vi "Run Tests.vi"(8 "error in (no error)":errorcluster, 10 "Test Cases":refnum<class "Test Case.lvclass">[](array[class]), 11 "LVUnit Test Executor in":refnum<class "LVUnit Test Executor.lvclass">) -> (0 "error out":errorcluster, 2 "Test Results":refnum<class "Test Result.lvclass">[](array[class]), 3 "LVUnit Test Executor out":refnum<class "LVUnit Test Executor.lvclass">)   [LabVIEW 2017, in "LVUnit Test Executor.lvclass"]
doc: "Runs the specified tests."
uses:
  LVUnit Test Executor.lvclass
  C:/Users/pasca/Projects/Home/lvunit/Test Executor/Test Executor.lvclass
  Test Case/Test Case.lvclass
  Test Result/Test Result.lvclass
  Test Outcome.ctl
  <vilib>/Utility/error.llb/DialogType.ctl
  Test Executor/Test Executor.lvclass/Test Executor.ctl
  Test Case/Test Case.lvclass/Test Case.ctl
  LVUnit Test Case/LVUnit Test Case.lvclass/LVUnit Test Case.ctl
  Test Result/Test Result.lvclass/Test Result.ctl
  Test Case/Get Path.vi
  LVUnit Test Case/Get JSON Data.vi
  Test Result/Set Outcome.vi
  Test Result/Set Failure Message.vi
  Test Result/Set Start Time.vi
  Test Result/Set End Time.vi
  Test Executor/Read Application.vi
  Test Executor/Read Result Queue.vi
  LVUnit Test Case/LVUnit Test Case.lvclass
  C:/Users/pasca/Projects/Home/lvunit/Test Case/Test Case.lvclass
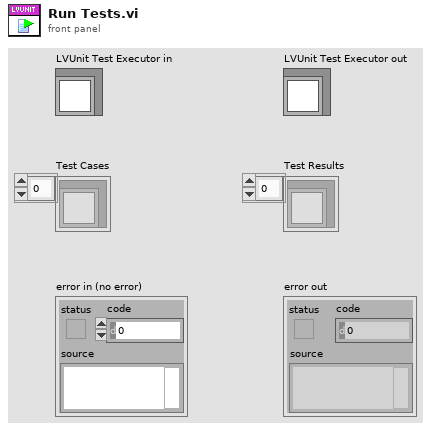
[diagram p1: front panel]
types:
  T1 = typedef "Test Outcome.ctl" = enum16{"None", "Passed", "Failed"}
  T2 = typedef "DialogType.ctl" = u16
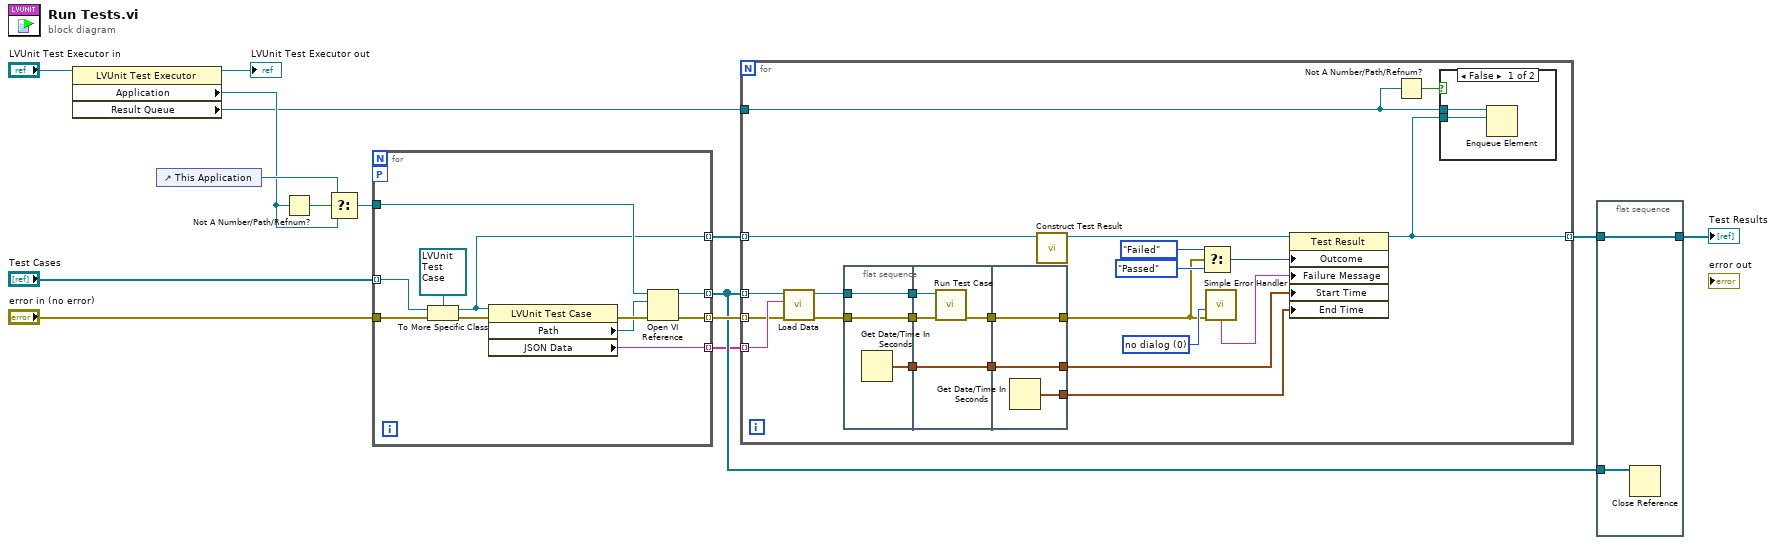
[diagram p0: block diagram]
diagram:
  n1 = property class="LVUnit Test Executor"(reference="LVUnit Test Executor in") -> (reference out=→"LVUnit Test Executor out":refnum<class "LVUnit Test Executor.lvclass">, "Application"=w11:refnum<vi>, "Result Queue"=w1:refnum<queue>)  [unwired: 1 in, 1 out]
  n2 = control-ref of="This Application"() -> (w12:refnum<vi>)
  n3 = Not A Number/Path/Refnum?(number/path/refnum=w11) -> (NaN/Path/Refnum?=w13:bool)
  n4 = Select(t=w12, s=w13, f=w11) -> (s? t:f=w8:refnum<vi>)
  n5 = for {
    tunnel: "Test Cases" -> [w22] mode=indexing
    tunnel: "error in (no error)" -> [w21]
    tunnel: w8 -> [w20]
    tunnel: [w19] -> w7 mode=indexing
    tunnel: [w18] -> w6 mode=indexing
    tunnel: [w17] -> w4 mode=indexing
    workers-P: _ -> [_]
    tunnel: [w16] -> w3 mode=indexing
    n6 = To More Specific Class(target class=refnum<class "LVUnit Test Case.lvclass"> refnum ("LVUnit Test Case.lvclass"), reference=w22, error in=w21) -> (specific class reference=w19:refnum<class "LVUnit Test Case.lvclass">, error out=w25:errorcluster)
    n7 = property class="LVUnit Test Case"(reference=w19, error in=w25) -> (error out=w24:errorcluster, "Path"=w23:path, "JSON Data"=w16:string)  [unwired: 1 out]
    n8 = Open VI Reference(application reference (local)=w20, vi path=w23, error in (no error)=w24) -> (vi reference=w17:refnum<vi>, error out=w18:errorcluster)  [unwired: 3 in]
  }
  n9 = for {
    tunnel: w7 -> [w30] mode=indexing
    tunnel: w6 -> [w40] mode=indexing
    tunnel: w4 -> [w42] mode=indexing
    tunnel: w3 -> [w41] mode=indexing
    tunnel: [w27] -> w2 mode=indexing
    tunnel: w1 -> [w28]
    w34 = T2 0 items=["no dialog", "OK message", "continue or stop message", "OK message + warnings", "continue/stop + warnings"] ("type of dialog (OK msg:1)")
    n10 = call "Load Data.vi"("error in (no error)"=w40, "JSON Data"=w41, "VI Reference"=w42) -> ("error out"=w49:errorcluster, "VI Refnum out"=w43:refnum<vi>)  [unwired: 7 in]
    n11 = flat-sequence {
      tunnel: w43 -> [w53]
      tunnel: w49 -> [w54]
      tunnel: [w54] -> w48
      tunnel: [w53] -> w47
      tunnel: [w52] -> w44
      tunnel: w48 -> [w57]
      tunnel: w47 -> [w56]
      tunnel: [w58] -> w46
      tunnel: [w55] -> w45
      tunnel: w44 -> [w55]
      tunnel: [w61] -> w33
      tunnel: w46 -> [w61]
      tunnel: [w60] -> w32
      tunnel: w45 -> [w60]
      tunnel: [w59] -> w31
      frame #0 {
        n12 = Get Date/Time In Seconds() -> (seconds since 1Jan1904=w52:timestamp)
      }
      frame #1 {
        n13 = call "Run Test Case.vi"("error in (no error)"=w57, "VI Refnum"=w56) -> ("error out"=w58:errorcluster)  [unwired: 8 in, 1 out]
      }
      frame #2 {
        n14 = Get Date/Time In Seconds() -> (seconds since 1Jan1904=w59:timestamp)
      }
    }
    n15 = call "Construct Test Result.vi"("Test Case"=w30) -> ("Test Result"=w39:refnum<class "Test Result.lvclass">)  [unwired: 9 in, 1 out]
    n16 = Select(t=Test_Outcome."Failed" ("Outcome"), s=w33, f=Test_Outcome."Passed" ("Outcome")) -> (s? t:f=w38:T1)
    n17 = call <vilib>:"Simple Error Handler.vi"("type of dialog (OK msg:1)"=w34, "error in (no error)"=w33) -> ("message"=w35:string)  [unwired: 3 in, 4 out]
    n18 = property class="Test Result"(reference=w39, "Outcome"=w38, "Failure Message"=w35, "Start Time"=w32, "End Time"=w31) -> (reference out=w27:refnum<class "Test Result.lvclass">)  [unwired: 1 in, 1 out]
    n19 = Not A Number/Path/Refnum?(number/path/refnum=w28) -> (NaN/Path/Refnum?=w29:bool)
    n20 = case shown="False" w29 {
      tunnel: w28 -> [w51 _]
      tunnel: w27 -> [w50 _]
      frame False {
        n21 = Enqueue Element(queue=w51, element=w50) -> ()  [unwired: 2 in, 3 out]
      }
      frame True {
      }
    }
  }
  n22 = flat-sequence {
    tunnel: [w62] -> w5
    tunnel: w4 -> [w63]
    tunnel: w2 -> [w62]
    frame #0 {
      n23 = Close Reference(reference=w63) -> ()  [unwired: 1 in, 1 out]
    }
  }
  "Test Results" <- w5
